vi "Create OneOf Accessors.vi"(8 "error in (no error)":errorcluster, 10 "MessageElementMetadata":T1, 11 "Oneof Class Ref In":refnum<vi>) -> (0 "error out":errorcluster, 3 "Oneof Class Ref Out":refnum<vi>)   [LabVIEW 2019, in "gRPC Template Creation Utility.lvlib"]
uses:
  gRPC Template Creation Utility.lvlib
  TypeDefs/Message Element Metadata (Scripting).ctl
  TypeDefs/Message Element Type.ctl
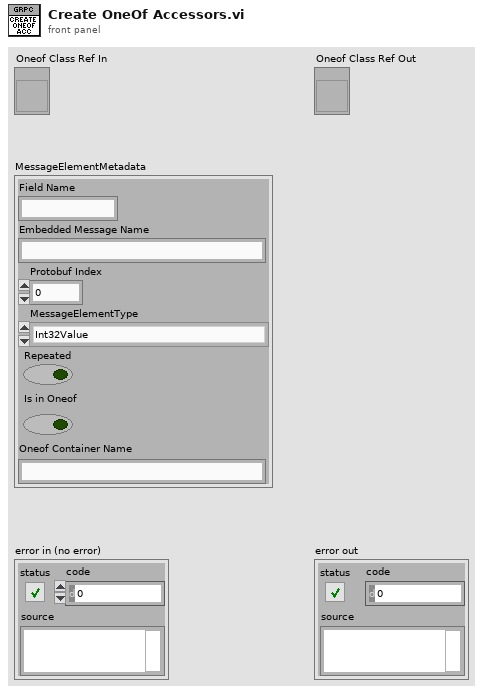
[diagram p1: front panel]
types:
  T1 = typedef "gRPC Template Creation Utility.lvlib/Message Element Metadata (Scripting).ctl" = cluster{"Field Name":string, "Embedded Message Name":string, "Protobuf Index":i32, "MessageElementType":T2, "Repeated":bool, "Is in Oneof":bool, "Oneof Container Name":string}
  T2 = typedef "gRPC Template Creation Utility.lvlib/Message Element Type.ctl" = enum32{"Int32Value", "FloatValue", "DoubleValue", "BoolValue", "StringValue", "MessageValue", "Int64Value", "UInt32Value", "UInt64Value", "EnumValue", "Bytes", "Fixed64", "Fixed32", "SFixed64", "SFixed32", "SInt64", "SInt32"}
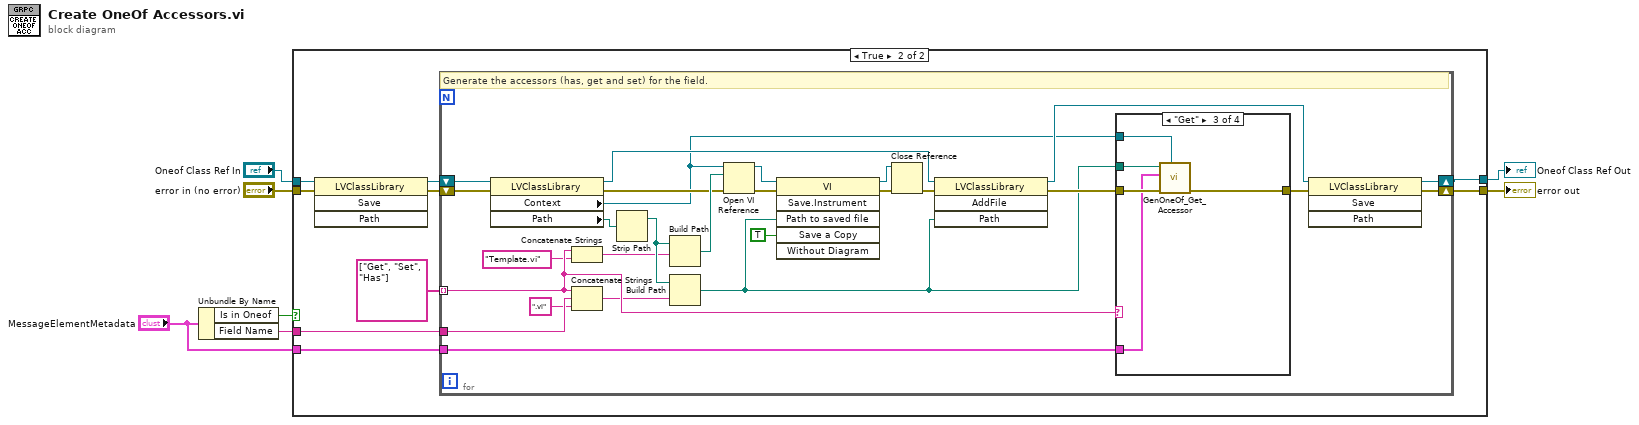
[diagram p0: block diagram]
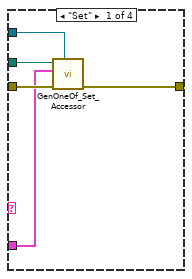
[diagram p3: hidden frame]
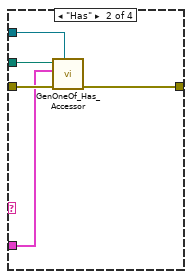
[diagram p4: hidden frame]
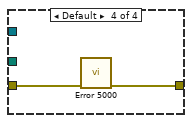
[diagram p5: hidden frame]
diagram:
  n1 = Unbundle By Name("MessageElementMetadata") -> ("Is in Oneof"=w5:bool, "Field Name"=w3:string)
  n2 = case shown="True" w5 {
    tunnel: "Oneof Class Ref In" -> [w8 w15]
    tunnel: w3 -> [_ w18]
    tunnel: [w9 w17] -> w4
    tunnel: "error in (no error)" -> [w9 w14]
    tunnel: [w8 w11] -> w2
    tunnel: "MessageElementMetadata" -> [_ w10]
    frame False {
    }
    frame True {
      n3 = invoke class="LVClassLibrary" method="Save"(reference=w15, error in=w14) -> (reference out=w12:refnum<vi>, error out=w13:errorcluster)  [unwired: 2 in, 2 out]
      n4 = for {
        tunnel: w18 -> [w44]
        shift-right: [w26] -> w17
        shift-left: w13 -> [w25]
        tunnel: string[] ["Get", "Set", "Has"] -> [w43] mode=indexing
        shift-right: [w23] -> w11
        shift-left: w12 -> [w45]
        tunnel: w10 -> [w19]
        # "Generate the accessors (has, get and set) for the field."
        n5 = property class="LVClassLibrary"(reference=w45, error in=w25) -> (reference out=w21:refnum<vi>, error out=w24:errorcluster, "Context"=w20:refnum<vi>, "Path"=w22:path)
        n6 = Concatenate Strings(w43, "Template.vi" ("Item Name")) -> (w37:string)
        n7 = Concatenate Strings(w43, w44, ".vi" ("string")) -> (w40:string)
        n8 = Strip Path(path=w22) -> (stripped path=w41:path)  [unwired: 1 out]
        n9 = Build Path(base path=w41, name or relative path=w37) -> (appended path=w34:path)
        n10 = Build Path(base path=w41, name or relative path=w40) -> (appended path=w35:path)
        n11 = Open VI Reference(application reference (local)=w20, vi path=w34, error in (no error)=w24) -> (vi reference=w32:refnum<vi>, error out=w33:errorcluster)  [unwired: 3 in]
        n12 = invoke class="VI" method="Save.Instrument"(reference=w32, error in=w33, "Path to saved file"=w35, "Save a Copy"=TRUE) -> (reference out=w29:refnum<vi>, error out=w30:errorcluster)  [unwired: 2 in, 4 out]
        n13 = Close Reference(reference=w29, error in (no error)=w30) -> (error out=w39:errorcluster)
        n14 = invoke class="LVClassLibrary" method="AddFile"(reference=w21, error in=w39, "Path"=w35) -> (reference out=w27:refnum<vi>, error out=w36:errorcluster)  [unwired: 1 in, 2 out]
        n15 = case shown="\"Get\"" w43 {
          tunnel: w36 -> [w50 w55 w60 w62]
          tunnel: w35 -> [w49 w54 w59 _]
          tunnel: [w48 w53 w58 w61] -> w28
          tunnel: w20 -> [w46 w51 w56 _]
          tunnel: w19 -> [w47 w52 w57 _]
          frame "Set" {
            # "Edit the VI"
            n16 = call "GenOneOf_Set_Accessor.vi"("application reference"=w46, "error in (no error)"=w50, "message element metadata"=w47, "path"=w49) -> ("error out"=w48:errorcluster)  [unwired: 7 in]
          }
          frame "Has" {
            # "Edit the VI"
            n17 = call "GenOneOf_Has_Accessor.vi"("application reference"=w51, "error in (no error)"=w55, "message element metadata"=w52, "path"=w54) -> ("error out"=w53:errorcluster)  [unwired: 7 in]
          }
          frame "Get" {
            # "Edit the VI"
            n18 = call "GenOneOf_Get_Accessor.vi"("application reference"=w56, "error in (no error)"=w60, "message element metadata"=w57, "path"=w59) -> ("error out"=w58:errorcluster)  [unwired: 7 in]
          }
          frame Default {
            n19 = call "Error 5000.vi"("error in (no error)"=w62) -> ("error out"=w61:errorcluster)  [unwired: 10 in]
          }
        }
        n20 = invoke class="LVClassLibrary" method="Save"(reference=w27, error in=w28) -> (reference out=w23:refnum<vi>, error out=w26:errorcluster)  [unwired: 2 in, 2 out]
      }
    }
  }
  "error out" <- w4
  "Oneof Class Ref Out" <- w2
